vi "order-analysis-unit-test.vi"(1 "Order Settings":T1={"Pulses per Rev"=1, "Trigger Level (V)"=2.5, "Hysteresis (V)"=0.5, "Slope"=enum."Rising", "Revs per Spectrum"=16, "Min Valid RPM"=300.0, "Orders"=[1.0, 2.0, 3.57, 4.0, 24.0], "Band Half-Width (order)"=0.19, "Max Order"=64.0, "Phase Bandwidth (order)"=0.25}, 4 "Noise (g rms)":dbl=0.01, 5 "Phases (deg)":dbl[](array[numeric])=[30.0, 0.0, 0.0, 0.0, 0.0], 6 "Orders":dbl[](array[numeric])=[1.0, 2.0, 3.57, 4.0, 24.0], 7 "Amplitudes (g pk)":dbl[](array[numeric])=[0.5, 0.2, 0.1, 0.05, 0.3], 8 "error in (no error)":errorcluster, 9 "Duration (s)":dbl=30.0, 10 "Ramps":T2(array[cluster]), 11 "Base RPM":dbl=3000.0) -> (0 "error out":errorcluster, 2 "True RPM":dbl[](array[numeric]), 3 "Values":dbl[][](array[numeric]))   [LabVIEW 2026]
doc: "Unit-test harness for OrderAnalysis.vi. Synthesises accel (sum of order sines, peak amplitudes, uniform noise) and a 1 ppr 0-5 V square tach (rising edge at shaft angle 0) for rpm(t) = Base RPM + sum of linear ramps, cuts it into 0.1 s blocks (5120 S @ 51.2 kS/s) and calls OrderAnalysis.vi block by block like FlexLogger Process.vi does (reset? TRUE on block 0, state in a shift register). Returns NUMERIC arrays only: Values [blocks x 12] in OrderAnalysis channel order, True RPM at each block centre."
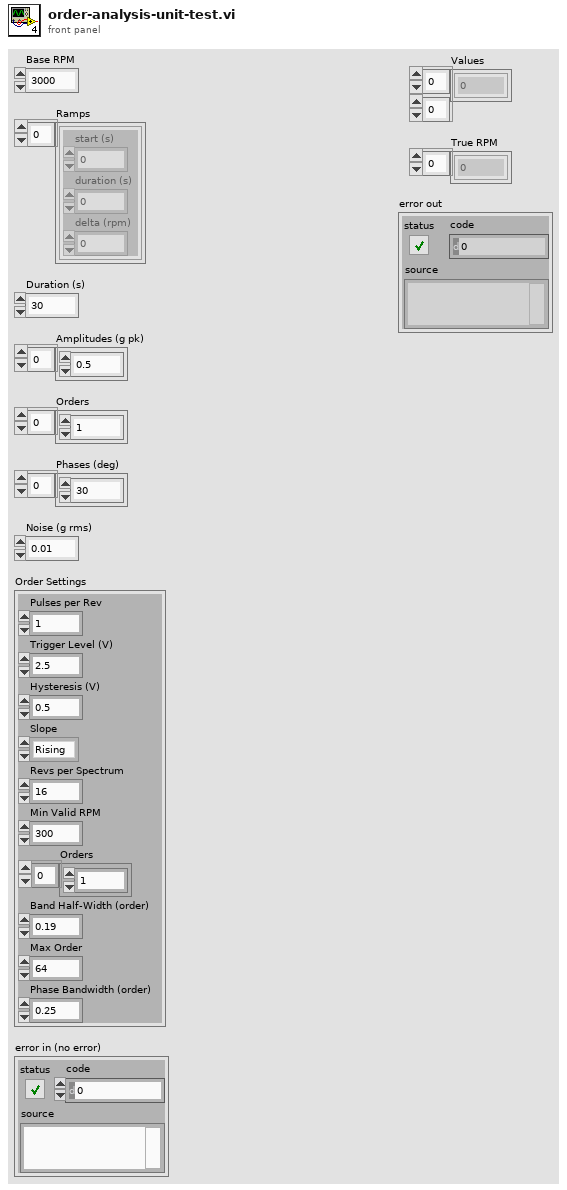
[diagram p1: front panel]
types:
  T1 = cluster{"Pulses per Rev":i32, "Trigger Level (V)":dbl, "Hysteresis (V)":dbl, "Slope":enum16{"Rising", "Falling"}, "Revs per Spectrum":i32, "Min Valid RPM":dbl, "Orders":dbl[], "Band Half-Width (order)":dbl, "Max Order":dbl, "Phase Bandwidth (order)":dbl}
  T2 = cluster{"start (s)":dbl, "duration (s)":dbl, "delta (rpm)":dbl}[]
  T3 = cluster{"Sample Count":dbl, "Last Time":dbl, "Last RPM":dbl, "Prev Time":dbl, "Anchor Time":dbl, "Anchor RPM":dbl, "RPM Rate":dbl, "Held Values":dbl[], "Has Spectrum":bool, "Was Valid":bool, "Acc SumSq":dbl, "Acc N":dbl}
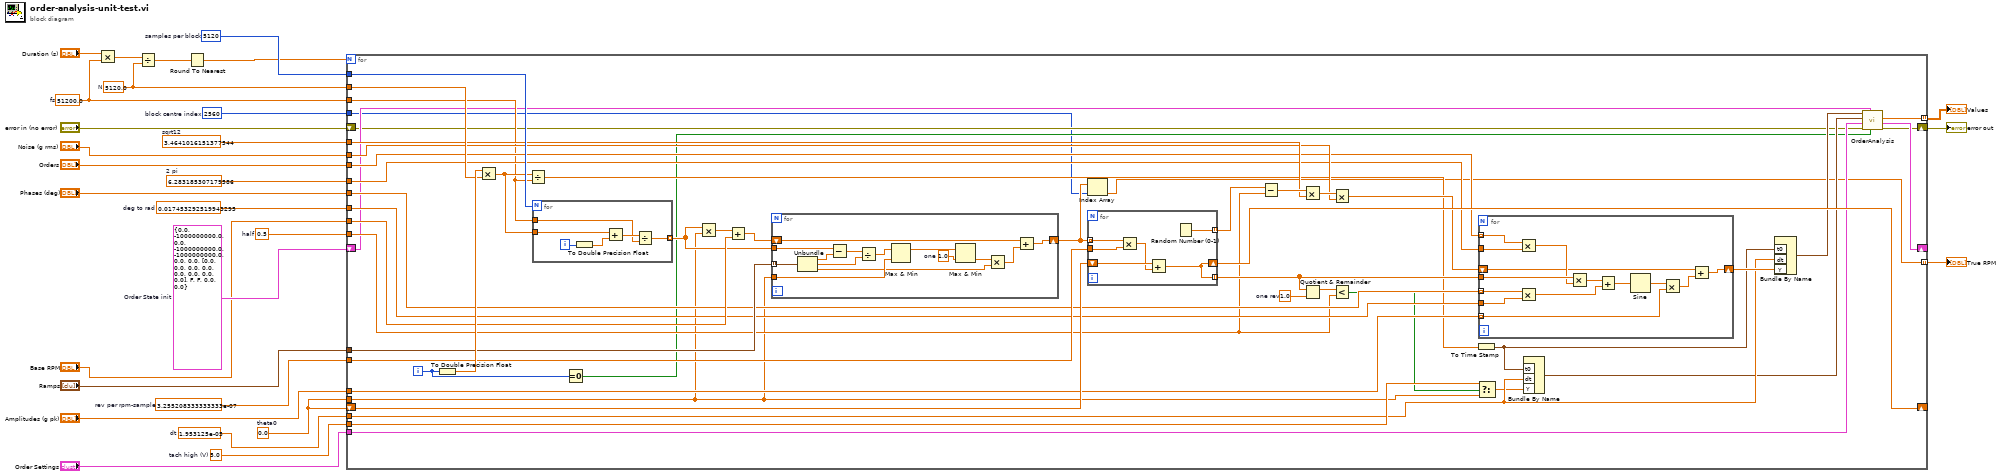
[diagram p0: block diagram]
diagram:
  w6 = 2560  # block centre index
  w7 = 5.0  # tach high (V)
  w8 = 6.283185307179586  # 2 pi
  w9 = 0.017453292519943295  # deg to rad
  w10 = 0.5  # half
  w11 = 3.4641016151377544  # sqrt12
  w12 = 1.953125e-05  # dt
  w13 = 3.255208333333333e-07  # rev per rpm-sample
  w5 = 0.0  # theta0
  w25 = T3 {"Sample Count"=0.0, "Last Time"=-1000000000.0, "Last RPM"=0.0, "Prev Time"=-1000000000.0, "Anchor Time"=-1000000000.0, "Anchor RPM"=0.0, "RPM Rate"=0.0, "Held Values"=[0.0, 0.0, 0.0, 0.0, 0.0, 0.0, 0.0, 0.0], "Has Spectrum"=FALSE, "Was Valid"=FALSE, "Acc SumSq"=0.0, "Acc N"=0.0}  # Order State init
  w14 = 5120.0  # N
  w15 = 5120  # samples per block
  w16 = 51200.0  # fs
  n1 = Multiply(x="Duration (s)", y=w16) -> (x*y=w27:dbl)
  n2 = Divide(x=w27, y=w14) -> (x/y=w26:dbl)
  n3 = Round To Nearest(number=w26) -> (nearest integer value=w4:dbl)
  n4 = for {
    N: w4 -> [_]
    shift-right: [w68] -> _
    shift-left: w5 -> [w67]
    shift-right: [w35] -> _
    shift-left: w25 -> [w38]
    shift-right: [w34] -> w1
    shift-left: "error in (no error)" -> [w36]
    tunnel: "Base RPM" -> [w73]
    tunnel: "Ramps" -> [w72]
    tunnel: "Amplitudes (g pk)" -> [w60]
    tunnel: "Orders" -> [w61]
    tunnel: "Phases (deg)" -> [w59]
    tunnel: "Noise (g rms)" -> [w62]
    tunnel: "Order Settings" -> [w39]
    tunnel: w16 -> [w47]
    tunnel: w15 -> [w75]
    tunnel: w14 -> [w76]
    tunnel: w13 -> [w69]
    tunnel: w12 -> [w43]
    tunnel: w11 -> [w64]
    tunnel: w10 -> [w52]
    tunnel: w9 -> [w57]
    tunnel: w8 -> [w58]
    tunnel: w7 -> [w51]
    tunnel: w6 -> [w32]
    tunnel: w5 -> [w49]
    tunnel: [w31] -> w3 mode=indexing
    tunnel: [w30] -> w2 mode=indexing
    i -> [w29]
    w54 = 1.0  # one rev
    n5 = To Double Precision Float(number=w29) -> (double precision float=w77:dbl)
    n6 = Multiply(x=w77, y=w76) -> (x*y=w48:dbl)
    n7 = Divide(x=w48, y=w47) -> (x/y=w46:dbl)
    n8 = for {
      N: w75 -> [_]
      tunnel: w48 -> [w117]
      tunnel: w47 -> [w114]
      tunnel: [w113] -> w71 mode=indexing
      i -> [w112]
      n9 = To Double Precision Float(number=w112) -> (double precision float=w116:dbl)
      n10 = Add(x=w117, y=w116) -> (x+y=w115:dbl)
      n11 = Divide(x=w115, y=w114) -> (x/y=w113:dbl)
    }
    n12 = Equal To 0?(x=w29) -> (x = 0?=w37:bool)
    n13 = Multiply(x=w71, y=w49) -> (x*y=w74:dbl[])
    n14 = Add(x=w74, y=w73) -> (x+y=w70:dbl[])
    n15 = for {
      tunnel: w72 -> [w111] mode=indexing
      tunnel: w71 -> [w110]
      tunnel: w49 -> [w105]
      shift-right: [w98] -> w33
      shift-left: w70 -> [w100]
      w103 = 1.0  # one
      n16 = Unbundle(w111) -> ("start (s)"=w109:dbl, "duration (s)"=w107:dbl, "delta (rpm)"=w101:dbl)
      n17 = Subtract(x=w110, y=w109) -> (x-y=w108:dbl[])
      n18 = Divide(x=w108, y=w107) -> (x/y=w106:dbl[])
      n19 = Max & Min(x=w106, y=w105) -> (max(x,y)=w104:dbl[])  [unwired: 1 out]
      n20 = Max & Min(x=w104, y=w103) -> (min(x,y)=w102:dbl[])  [unwired: 1 out]
      n21 = Multiply(x=w102, y=w101) -> (x*y=w99:dbl[])
      n22 = Add(x=w100, y=w99) -> (x+y=w98:dbl[])
    }
    n23 = Index Array(array=w33, index=w32) -> (element=w30:dbl)
    n24 = for {
      tunnel: w33 -> [w97] mode=indexing
      tunnel: w69 -> [w96]
      shift-right: [w93] -> w68
      shift-left: w67 -> [w95]
      tunnel: [w93] -> w55 mode=indexing
      tunnel: [w92] -> w66 mode=indexing
      n25 = Multiply(x=w97, y=w96) -> (x*y=w94:dbl)
      n26 = Add(x=w95, y=w94) -> (x+y=w93:dbl)
      n27 = Random Number (0-1)() -> (number: 0 to 1=w92:dbl)
    }
    n28 = Subtract(x=w66, y=w52) -> (x-y=w65:dbl[])
    n29 = Multiply(x=w65, y=w64) -> (x*y=w63:dbl[])
    n30 = Quotient & Remainder(x=w55, y=w54) -> (x-y*floor(x/y)=w53:dbl[])  [unwired: 1 out]
    n31 = Multiply(x=w63, y=w62) -> (x*y=w56:dbl[])
    n32 = Less?(x=w53, y=w52) -> (x < y?=w50:bool[])
    n33 = To Time Stamp(1:w46) -> (0:w44:timestamp)
    n34 = Select(t=w51, s=w50, f=w49) -> (s? t:f=w42:dbl)
    n35 = for {
      tunnel: w61 -> [w91] mode=indexing
      tunnel: w60 -> [w81] mode=indexing
      tunnel: w59 -> [w87] mode=indexing
      tunnel: w55 -> [w89]
      tunnel: w58 -> [w90]
      tunnel: w57 -> [w86]
      shift-right: [w78] -> w45
      shift-left: w56 -> [w80]
      n36 = Multiply(x=w91, y=w90) -> (x*y=w88:dbl)
      n37 = Multiply(x=w87, y=w86) -> (x*y=w84:dbl)
      n38 = Multiply(x=w89, y=w88) -> (x*y=w85:dbl[])
      n39 = Add(x=w85, y=w84) -> (x+y=w83:dbl[])
      n40 = Sine(x=w83) -> (sin(x)=w82:dbl[])
      n41 = Multiply(x=w82, y=w81) -> (x*y=w79:dbl[])
      n42 = Add(x=w80, y=w79) -> (x+y=w78:dbl[])
    }
    n43 = Bundle By Name("t0"=w44, "dt"=w43, "Y"=w42) -> (w40:waveform(dbl))  [unwired: 1 in]
    n44 = Bundle By Name("t0"=w44, "dt"=w43, "Y"=w45) -> (w41:waveform(dbl))  [unwired: 1 in]
    n45 = call "OrderAnalysis.vi"("reset? (F)"=w37, "Order State in"=w38, "error in (no error)"=w36, "Order Settings"=w39, "Tach In"=w40, "Accel In"=w41) -> ("error out"=w34:errorcluster, "Order State out"=w35:T3, "Order Values"=w31:dbl[])  [unwired: 2 in, 1 out]
  }
  "Values" <- w3
  "True RPM" <- w2
  "error out" <- w1
